vi "RemoteVI Hover Navigate.vi"(0 "hWnd":u64, 5 "menu":T2, 7 "state":T1, 9 "now":u32, 11 "error in":errorcluster) -> (4 "state out":T1, 15 "error out":errorcluster)   [LabVIEW 2020, in "RemoteVI.lvlib"]
doc: "Applies the remote pointer to the deepest open LabVIEW menu, like a local hover: RemoteVI Highlight Menu Row.vi moves the menu's highlight onto the item under the pointer (state.y, a logical screen y, taken relative to menu.y) with VK_DOWN / VK_UP - no cursor and no window is moved. The menu pointer state is updated: navigated TRUE; menu, top and hit from the result; when the highlighted band moved to another item (or another menu) row since becomes now and dwelled FALSE, so the dwell timer of RemoteVI Menu Hover.vi starts again; when the window showed no highlight even after the probe key it is no keyboard menu and becomes state.plain (the mouse path handles it). No VI Server call."
uses:
  RemoteVI.lvlib
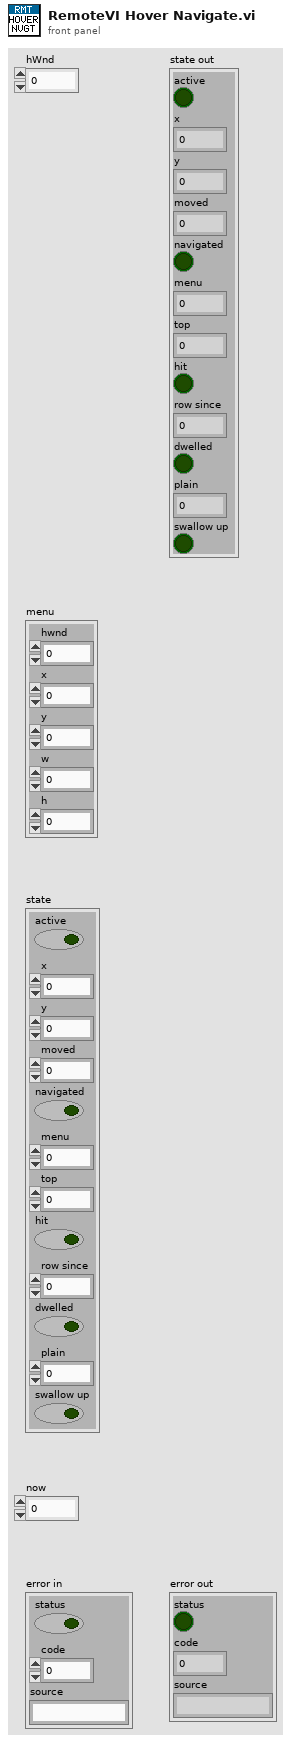
[diagram p1: front panel]
types:
  T1 = cluster{"active":bool, "x":i32, "y":i32, "moved":u32, "navigated":bool, "menu":u64, "top":i32, "hit":bool, "row since":u32, "dwelled":bool, "plain":u64, "swallow up":bool}
  T2 = cluster{"hwnd":u64, "x":i32, "y":i32, "w":i32, "h":i32}
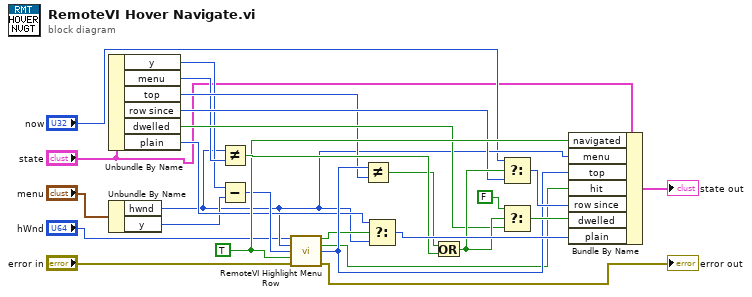
[diagram p0: block diagram]
diagram:
  w15 = TRUE
  n1 = Unbundle By Name("state") -> ("y"=w8:i32, "menu"=w9:u64, "top"=w10:i32, "row since"=w11:u32, "dwelled"=w12:bool, "plain"=w13:u64)
  n2 = Unbundle By Name("menu") -> ("hwnd"=w6:u64, "y"=w7:i32)
  n3 = Not Equal?(x=w6, y=w9) -> (x != y?=w22:bool)
  n4 = Subtract(x=w8, y=w7) -> (x-y=w14:i32)
  n5 = call "RemoteVI Highlight Menu Row.vi"("hWnd"="hWnd", "menu"=w6, "y"=w14, "probe?"=w15, "error in"="error in") -> ("keyed?"=w17:bool, "hit?"=w18:bool, "top"=w19:i32, "error out"=→"error out":errorcluster)  [unwired: 6 in, 1 out]
  n6 = Not Equal?(x=w19, y=w10) -> (x != y?=w21:bool)
  n7 = Select(t=w13, s=w17, f=w6) -> (s? t:f=w26:u64)
  n8 = Or(x=w21, y=w22) -> (x .or. y?=w23:bool)
  n9 = Select(t="now", s=w23, f=w11) -> (s? t:f=w24:u32)
  n10 = Select(t=FALSE, s=w23, f=w12) -> (s? t:f=w25:bool)
  n11 = Bundle By Name(cluster="state", "navigated"=w15, "menu"=w6, "top"=w19, "hit"=w18, "row since"=w24, "dwelled"=w25, "plain"=w26) -> (→"state out":T1)
